vi "before and after.vi"(8 "エラー入力":errorcluster, 9 "after":string, 11 "Before":string) -> (0 "エラー出力":errorcluster, 3 "Anal Time":string)   [LabVIEW 2018]
panel:
  out "数値 8":i32
  out "数値 7":i32
  out "H":i32
  out "M":i32
  out "S":i32
  out "x - y":i32
  out "結果 2":i32
  out "数値 6":i32
  out "数値 5":i32
  out "数値 4":i32
  out "部分文字列の後 2":string
  out "部分文字列の前 4":string
  out "部分文字列の前 3":string
  out "結果":i32
  out "数値 3":i32
  out "数値 2":i32
  out "数値":i32
  out "部分文字列の後":string
  out "部分文字列の前 2":string
  out "部分文字列の前":string
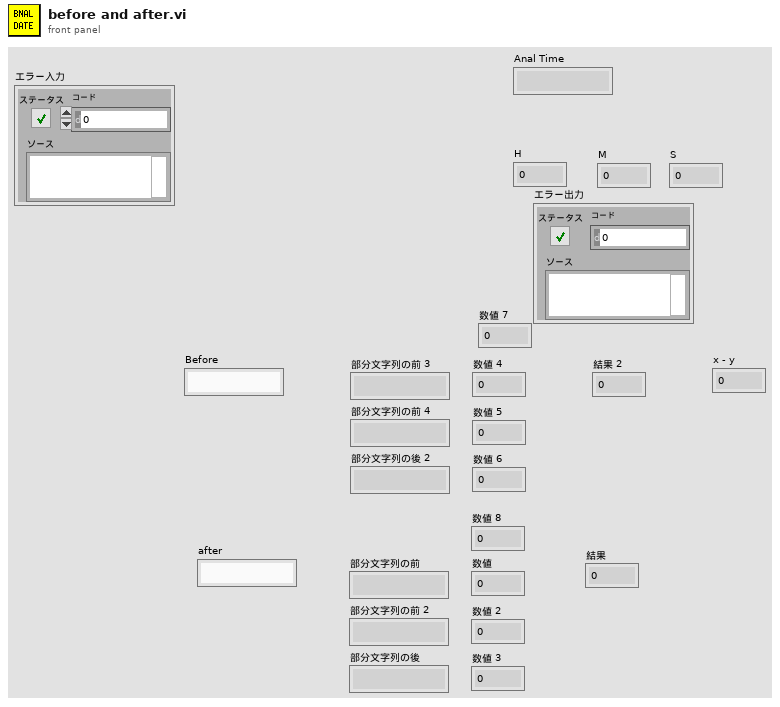
[diagram p1: front panel]
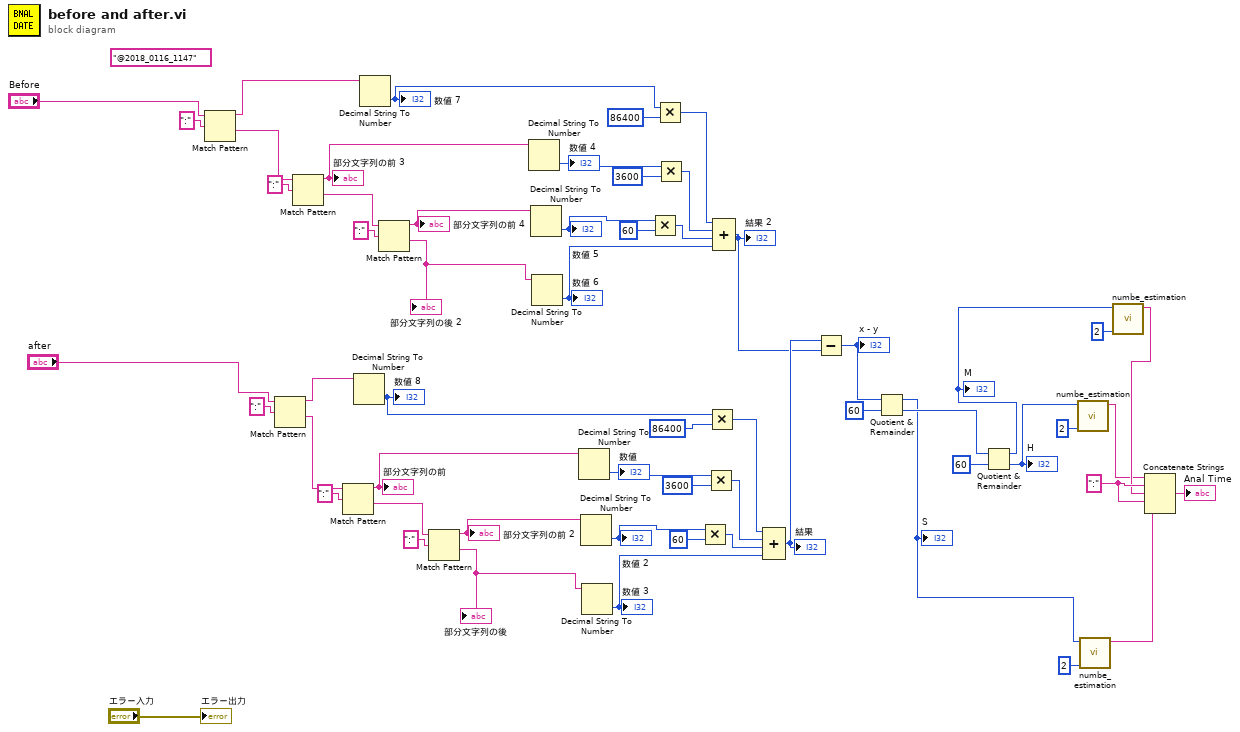
[diagram p0: block diagram]
diagram:
  (unwired) "@2018_0116_1147" ("Date")
  w26 = ":" ("文字列")
  n1 = Match Pattern(string="Before", regular expression=":" ("検索文字列")) -> (before substring=w9:string, after substring=w10:string)  [unwired: 1 in, 2 out]
  n2 = Match Pattern(string="after", regular expression=":" ("検索文字列")) -> (before substring=w8:string, after substring=w13:string)  [unwired: 1 in, 2 out]
  n3 = Match Pattern(string=w10, regular expression=":" ("検索文字列")) -> (before substring=w42:string, after substring=w43:string)  [unwired: 1 in, 2 out]
  "部分文字列の前 3" <- w42
  n4 = Match Pattern(string=w13, regular expression=":" ("検索文字列")) -> (before substring=w55:string, after substring=w56:string)  [unwired: 1 in, 2 out]
  "部分文字列の前" <- w55
  n5 = Decimal String To Number(string=w8) -> (number=w2:i32)  [unwired: 2 in, 1 out]
  "数値 8" <- w2
  n6 = Decimal String To Number(string=w9) -> (number=w3:i32)  [unwired: 2 in, 1 out]
  "数値 7" <- w3
  n7 = Match Pattern(string=w43, regular expression=":" ("検索文字列")) -> (before substring=w41:string, after substring=w40:string)  [unwired: 1 in, 2 out]
  "部分文字列の前 4" <- w41
  "部分文字列の後 2" <- w40
  n8 = Match Pattern(string=w56, regular expression=":" ("検索文字列")) -> (before substring=w54:string, after substring=w53:string)  [unwired: 1 in, 2 out]
  "部分文字列の前 2" <- w54
  "部分文字列の後" <- w53
  n9 = Decimal String To Number(string=w42) -> (number=w36:i32)  [unwired: 2 in, 1 out]
  "数値 4" <- w36
  n10 = Decimal String To Number(string=w41) -> (number=w39:i32)  [unwired: 2 in, 1 out]
  "数値 5" <- w39
  n11 = Decimal String To Number(string=w40) -> (number=w33:i32)  [unwired: 2 in, 1 out]
  "数値 6" <- w33
  n12 = Decimal String To Number(string=w55) -> (number=w49:i32)  [unwired: 2 in, 1 out]
  "数値" <- w49
  n13 = Decimal String To Number(string=w54) -> (number=w52:i32)  [unwired: 2 in, 1 out]
  "数値 2" <- w52
  n14 = Decimal String To Number(string=w53) -> (number=w46:i32)  [unwired: 2 in, 1 out]
  "数値 3" <- w46
  n15 = Multiply(x=w39, y=60) -> (x*y=w34:i32)
  n16 = Multiply(x=w3, y=86400) -> (x*y=w6:i32)
  n17 = Multiply(x=w36, y=3600) -> (x*y=w35:i32)
  n18 = Multiply(x=w52, y=60) -> (x*y=w47:i32)
  n19 = Multiply(x=w49, y=3600) -> (x*y=w48:i32)
  n20 = Multiply(x=w2, y=86400) -> (x*y=w5:i32)
  n21 = Compound Arithmetic op=ADD(w6, w35, w34, w33) -> (w31:i32)
  "結果 2" <- w31
  n22 = Compound Arithmetic op=ADD(w5, w48, w47, w46) -> (w32:i32)
  "結果" <- w32
  n23 = Subtract(x=w32, y=w31) -> (x-y=w30:i32)
  "x - y" <- w30
  n24 = Quotient & Remainder(x=w30, y=60) -> (x-y*floor(x/y)=w22:i32, floor(x/y)=w27:i32)
  "S" <- w22
  n25 = Quotient & Remainder(x=w27, y=60) -> (x-y*floor(x/y)=w20:i32, floor(x/y)=w17:i32)
  "M" <- w20
  "H" <- w17
  n26 = call "numbe_estimation.vi"("桁数"=2, "数値"=w17) -> ("数値文字列"=w16:string)  [unwired: 9 in]
  n27 = call "numbe_estimation.vi"("桁数"=2, "数値"=w22) -> ("数値文字列"=w21:string)  [unwired: 9 in]
  n28 = call "numbe_estimation.vi"("桁数"=2, "数値"=w20) -> ("数値文字列"=w19:string)  [unwired: 9 in]
  n29 = Concatenate Strings(w16, w26, w19, w26, w21) -> (→"Anal Time":string)
  "エラー出力" <- "エラー入力"
